vi "Notify Stop.vi"() -> ()   [LabVIEW 2020]
doc: "Dev helper: sends a notification on RemoteVI:<port> (stops that server loop) without waiting."
panel:
  out "error out":errorcluster
  in  "port":u16=8089
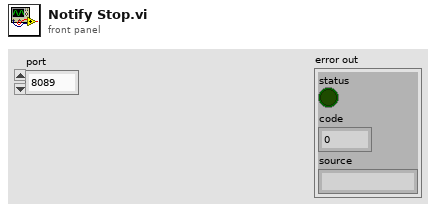
[diagram p1: front panel]
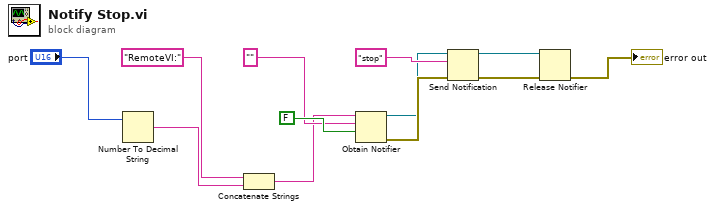
[diagram p0: block diagram]
diagram:
  n1 = Number To Decimal String(number="port") -> (decimal integer string=w3:string)  [unwired: 1 in]
  n2 = Concatenate Strings("RemoteVI:", w3) -> (w4:string)
  n3 = Obtain Notifier(name (unnamed)=w4, notification data type="", create if not found? (T)=FALSE) -> (notifier out=w7:refnum<notifier>, error out=w8:errorcluster)  [unwired: 1 in, 1 out]
  n4 = Send Notification(notification="stop", notifier=w7, error in (no error)=w8) -> (notifier out=w10:refnum<notifier>, error out=w11:errorcluster)
  n5 = Release Notifier(notifier=w10, error in (no error)=w11) -> (error out=→"error out":errorcluster)  [unwired: 1 in, 2 out]
